vi "Trade.generated.vi"(11 "buffer.in":u64[](array[numeric])=[0, 0, 0, 0, 0, 0, 0, 0, 0]) -> (3 "OrderBook.Command":T1)   [LabVIEW 2020]
doc: "Cboe PITCH Trade (0x2A long, 0x2B short, 0x30 expanded) -> orderbook.command: type Trade (enum value 10, add Trade=10 and Unsupported=11 to orderbook.command.type.ctl), orderId, side, quantity, symbol (8 chars, space padded), price, nanoseconds. Short price x100 so all prices have 4 implied decimals."
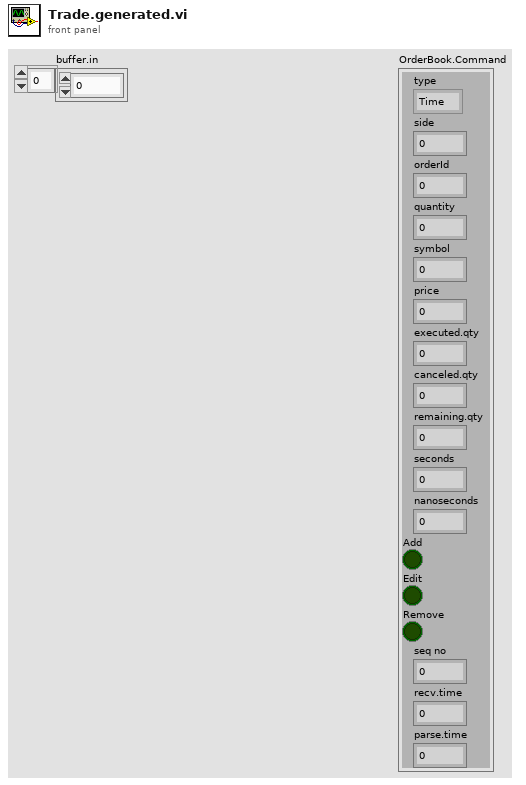
[diagram p1: front panel]
types:
  T1 = cluster{"type":enum8{"Time", "AddOrder", "OrderExecuted", "OrderExecutedAtPrice", "ReduceSize", "ModifyOrder", "DeleteOrder", "Get.Everything", "Get.All.Orders", "Get.Top", "Trade", "Unsupported"}, "side":u8, "orderId ":u64, "quantity":u32, "symbol":u64, "price":u64, "executed.qty":u32, "canceled.qty":u32, "remaining.qty":u32, "seconds":u64, "nanoseconds":u64, "Add":bool, "Edit":bool, "Remove":bool, "seq no":u32, "recv.time":u64, "parse.time":u64}
  T2 = enum8{"Time", "AddOrder", "OrderExecuted", "OrderExecutedAtPrice", "ReduceSize", "ModifyOrder", "DeleteOrder", "Get.Everything", "Get.All.Orders", "Get.Top", "Trade", "Unsupported"}
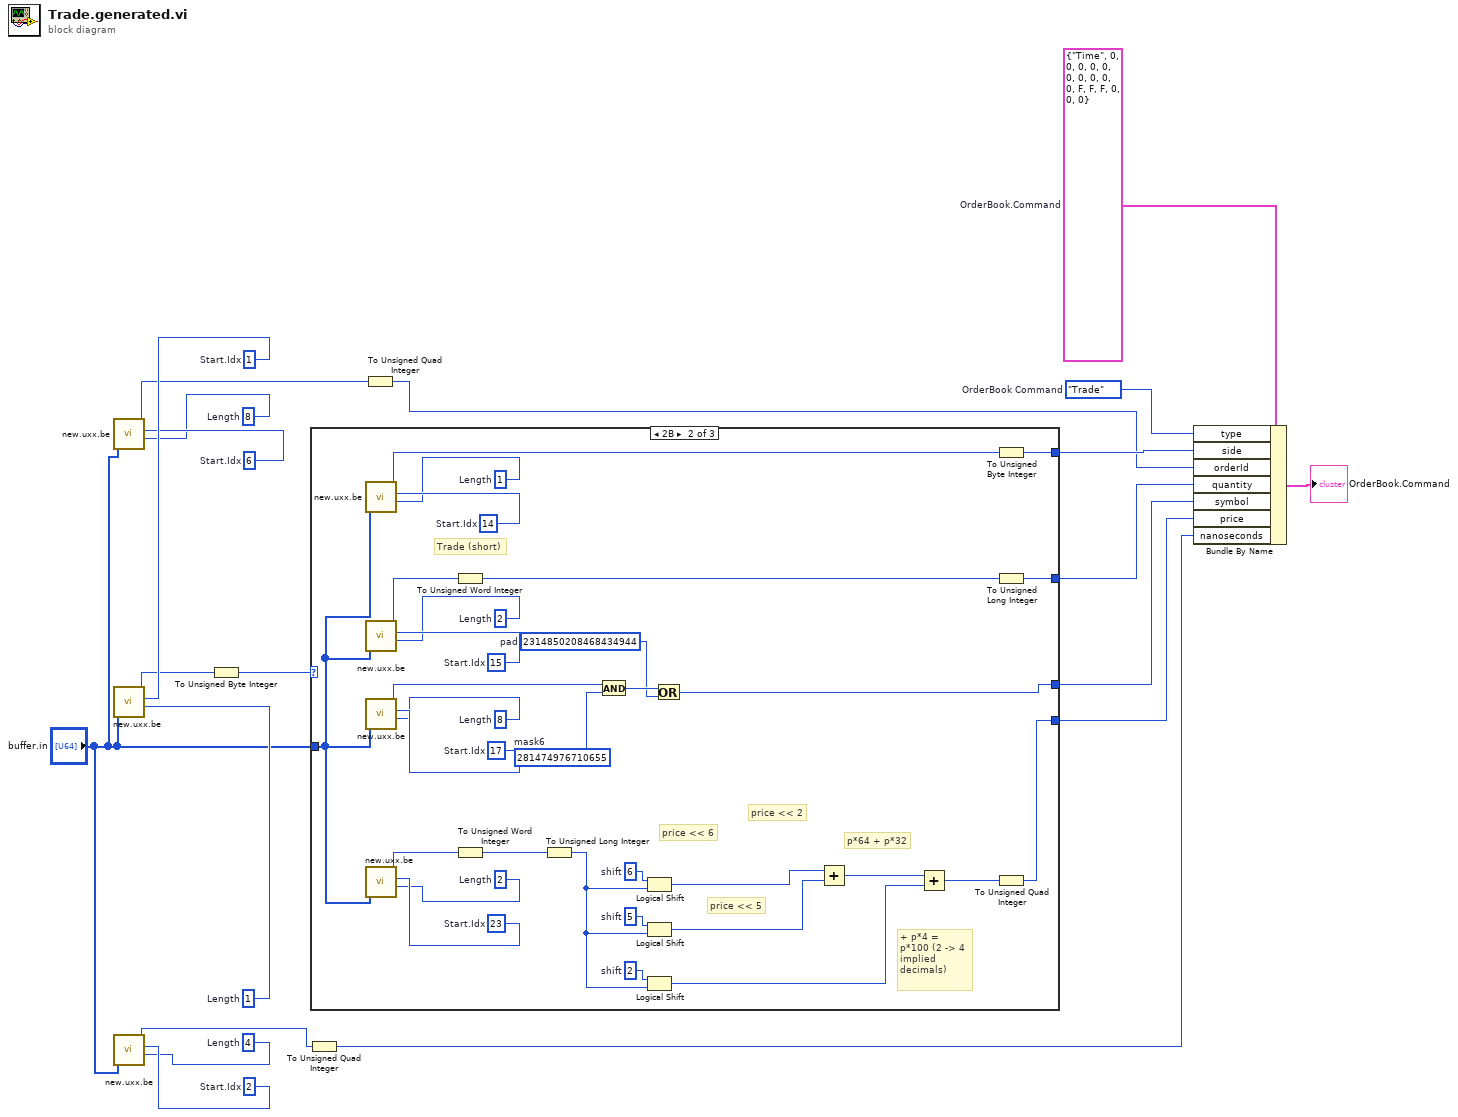
[diagram p0: block diagram]
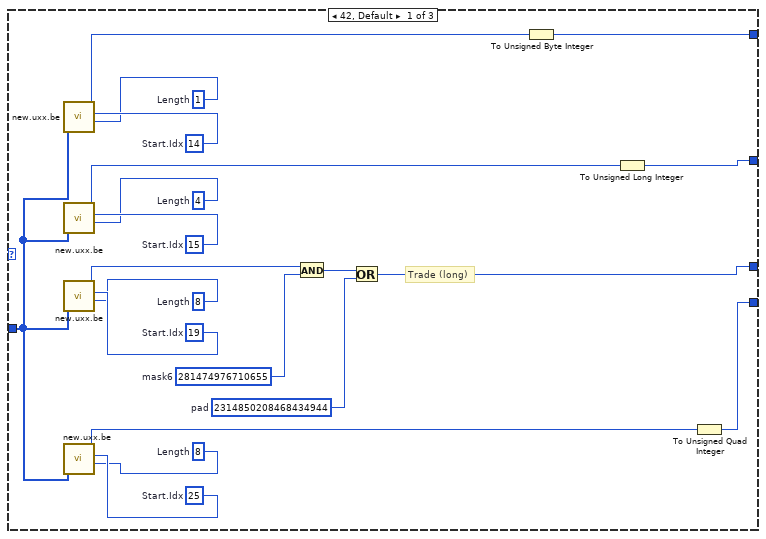
[diagram p2: hidden frame]
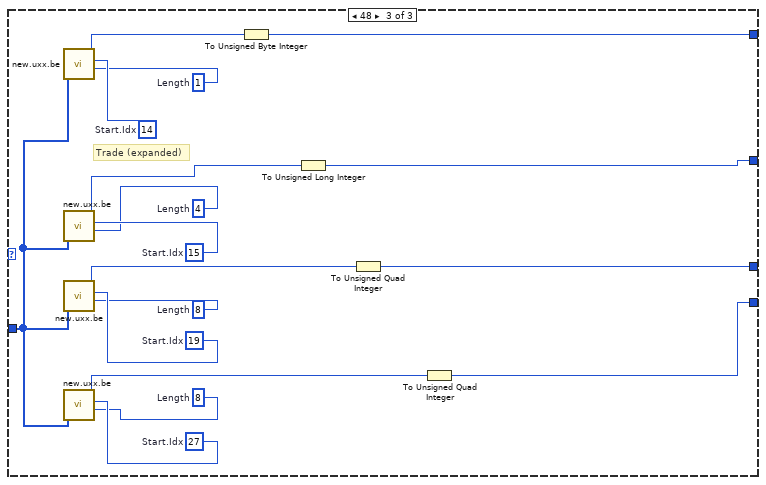
[diagram p3: hidden frame]
diagram:
  w13 = u8 8  # Length
  w14 = u8 6  # Start.Idx
  w16 = u8 4  # Length
  w17 = u8 2  # Start.Idx
  w19 = u8 1  # Length
  w20 = u8 1  # Start.Idx
  w9 = T2."Trade"  # OrderBook Command
  w2 = T1 {"type"=enum."Time", "side"=0, "orderId "=0, "quantity"=0, "symbol"=0, "price"=0, "executed.qty"=0, "canceled.qty"=0, "remaining.qty"=0, "seconds"=0, "nanoseconds"=0, "Add"=FALSE, "Edit"=FALSE, "Remove"=FALSE, "seq no"=0, "recv.time"=0, "parse.time"=0}  # OrderBook.Command
  n1 = call "new.uxx.be.vi"("buffer (U64)"="buffer.in", "Start.Idx"=w14, "Length"=w13) -> ("Out.Value U64"=w12:u64)  [unwired: 7 in]
  n2 = call "new.uxx.be.vi"("buffer (U64)"="buffer.in", "Start.Idx"=w20, "Length"=w19) -> ("Out.Value U64"=w18:u64)  [unwired: 7 in]
  n3 = call "new.uxx.be.vi"("buffer (U64)"="buffer.in", "Start.Idx"=w17, "Length"=w16) -> ("Out.Value U64"=w15:u64)  [unwired: 7 in]
  n4 = To Unsigned Byte Integer(number=w18) -> (unsigned 8bit integer=w10:u8)
  n5 = To Unsigned Quad Integer(1:w15) -> (0:w3:u64)
  n6 = case shown="2B" w10 {
    tunnel: "buffer.in" -> [w28 w58 w79]
    tunnel: [w24 w44 w75] -> w8
    tunnel: [w23 w43 w74] -> w6
    tunnel: [w22 w42 w73] -> w5
    tunnel: [w21 w41 w72] -> w4
    frame 42, Default {
      w26 = u8 8  # Length
      w27 = u8 25  # Start.Idx
      w29 = u64 2314850208468434944  # pad
      w31 = u64 281474976710655  # mask6
      w33 = u8 8  # Length
      w34 = u8 19  # Start.Idx
      w36 = u8 4  # Length
      w37 = u8 15  # Start.Idx
      w39 = u8 1  # Length
      w40 = u8 14  # Start.Idx
      # "Trade (long)"
      n7 = call "new.uxx.be.vi"("buffer (U64)"=w28, "Start.Idx"=w40, "Length"=w39) -> ("Out.Value U64"=w38:u64)  [unwired: 7 in]
      n8 = call "new.uxx.be.vi"("buffer (U64)"=w28, "Start.Idx"=w37, "Length"=w36) -> ("Out.Value U64"=w35:u64)  [unwired: 7 in]
      n9 = call "new.uxx.be.vi"("buffer (U64)"=w28, "Start.Idx"=w34, "Length"=w33) -> ("Out.Value U64"=w32:u64)  [unwired: 7 in]
      n10 = call "new.uxx.be.vi"("buffer (U64)"=w28, "Start.Idx"=w27, "Length"=w26) -> ("Out.Value U64"=w25:u64)  [unwired: 7 in]
      n11 = And(x=w32, y=w31) -> (x .and. y?=w30:u64)
      n12 = Or(x=w30, y=w29) -> (x .or. y?=w22:u64)
      n13 = To Unsigned Byte Integer(number=w38) -> (unsigned 8bit integer=w24:u8)
      n14 = To Unsigned Long Integer(number=w35) -> (unsigned 32bit integer=w23:u32)
      n15 = To Unsigned Quad Integer(1:w25) -> (0:w21:u64)
    }
    frame 43 {
      w51 = i16 2  # shift
      w52 = i16 5  # shift
      w53 = i16 6  # shift
      w56 = u8 2  # Length
      w57 = u8 23  # Start.Idx
      w59 = u64 2314850208468434944  # pad
      w61 = u64 281474976710655  # mask6
      w63 = u8 8  # Length
      w64 = u8 17  # Start.Idx
      w67 = u8 2  # Length
      w68 = u8 15  # Start.Idx
      w70 = u8 1  # Length
      w71 = u8 14  # Start.Idx
      # "+ p*4 = p*100 (2 -> 4 implied decimals)"
      # "p*64 + p*32"
      # "price << 2"
      # "price << 5"
      # "price << 6"
      # "Trade (short)"
      n16 = call "new.uxx.be.vi"("buffer (U64)"=w58, "Start.Idx"=w71, "Length"=w70) -> ("Out.Value U64"=w69:u64)  [unwired: 7 in]
      n17 = call "new.uxx.be.vi"("buffer (U64)"=w58, "Start.Idx"=w68, "Length"=w67) -> ("Out.Value U64"=w66:u64)  [unwired: 7 in]
      n18 = call "new.uxx.be.vi"("buffer (U64)"=w58, "Start.Idx"=w64, "Length"=w63) -> ("Out.Value U64"=w62:u64)  [unwired: 7 in]
      n19 = call "new.uxx.be.vi"("buffer (U64)"=w58, "Start.Idx"=w57, "Length"=w56) -> ("Out.Value U64"=w55:u64)  [unwired: 7 in]
      n20 = To Unsigned Word Integer(number=w66) -> (unsigned 16bit integer=w65:u16)
      n21 = To Unsigned Word Integer(number=w55) -> (unsigned 16bit integer=w54:u16)
      n22 = To Unsigned Long Integer(number=w54) -> (unsigned 32bit integer=w50:u32)
      n23 = And(x=w62, y=w61) -> (x .and. y?=w60:u64)
      n24 = Logical Shift(y=w53, x=w50) -> (x << y=w49:u32)
      n25 = Logical Shift(y=w52, x=w50) -> (x << y=w48:u32)
      n26 = Logical Shift(y=w51, x=w50) -> (x << y=w46:u32)
      n27 = Or(x=w60, y=w59) -> (x .or. y?=w42:u64)
      n28 = Add(x=w49, y=w48) -> (x+y=w47:u32)
      n29 = Add(x=w47, y=w46) -> (x+y=w45:u32)
      n30 = To Unsigned Byte Integer(number=w69) -> (unsigned 8bit integer=w44:u8)
      n31 = To Unsigned Long Integer(number=w65) -> (unsigned 32bit integer=w43:u32)
      n32 = To Unsigned Quad Integer(1:w45) -> (0:w41:u64)
    }
    frame 48 {
      w77 = u8 8  # Length
      w78 = u8 27  # Start.Idx
      w81 = u8 8  # Length
      w82 = u8 19  # Start.Idx
      w84 = u8 4  # Length
      w85 = u8 15  # Start.Idx
      w87 = u8 1  # Length
      w88 = u8 14  # Start.Idx
      # "Trade (expanded)"
      n33 = call "new.uxx.be.vi"("buffer (U64)"=w79, "Start.Idx"=w88, "Length"=w87) -> ("Out.Value U64"=w86:u64)  [unwired: 7 in]
      n34 = call "new.uxx.be.vi"("buffer (U64)"=w79, "Start.Idx"=w85, "Length"=w84) -> ("Out.Value U64"=w83:u64)  [unwired: 7 in]
      n35 = call "new.uxx.be.vi"("buffer (U64)"=w79, "Start.Idx"=w82, "Length"=w81) -> ("Out.Value U64"=w80:u64)  [unwired: 7 in]
      n36 = call "new.uxx.be.vi"("buffer (U64)"=w79, "Start.Idx"=w78, "Length"=w77) -> ("Out.Value U64"=w76:u64)  [unwired: 7 in]
      n37 = To Unsigned Byte Integer(number=w86) -> (unsigned 8bit integer=w75:u8)
      n38 = To Unsigned Long Integer(number=w83) -> (unsigned 32bit integer=w74:u32)
      n39 = To Unsigned Quad Integer(1:w80) -> (0:w73:u64)
      n40 = To Unsigned Quad Integer(1:w76) -> (0:w72:u64)
    }
  }
  n41 = To Unsigned Quad Integer(1:w12) -> (0:w7:u64)
  n42 = Bundle By Name(cluster=w2, "type"=w9, "side"=w8, "orderId"=w7, "quantity"=w6, "symbol"=w5, "price"=w4, "nanoseconds"=w3) -> (→"OrderBook.Command":T1)
